vi "Log Status.vi"(7 "Context ID":u32, 8 "error in":errorcluster, 9 "Action":T1, 10 "Socket Counter":u32, 11 "Context Counter":u32) -> (0 "error out":errorcluster)   [LabVIEW 2019, in "RemoteControl.ZMQ.lvlib" / "ZMQ.ContextManager.lvlib"]
uses:
  ZMQ.ContextManager.lvlib
  Typedefs/Action--enum.ctl
  <vilib>/Utility/sysdir.llb/System Directory Type.ctl
  <vilib>/Utility/file.llb/Write Delimited Spreadsheet (string).vi
  <vilib>/Utility/config.llb/Read Key (Boolean).vi
  <vilib>/Utility/config.llb/Write Key (Boolean).vi
  <vilib>/Utility/config.llb/NI_LVConfig.lvlib
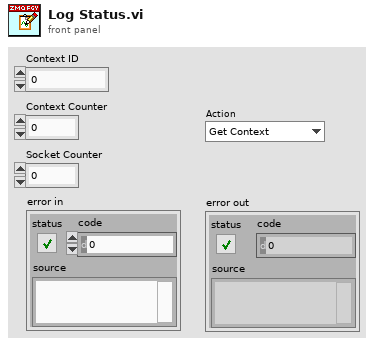
[diagram p1: front panel]
types:
  T1 = typedef "RemoteControl.ZMQ.lvlib/ZMQ.ContextManager.lvlib/Action--enum.ctl" = enum16{"Get Context", "Release Context", "Socket Opened", "Socket Closed", "Force Cleanup", "Set Context", "Retire If Idle"}
  T2 = typedef "System Directory Type.ctl" = i32
  T3 = typedef "NI_LVConfig.lvlib/Config Data RefNum.ctl" = refnum<k1>
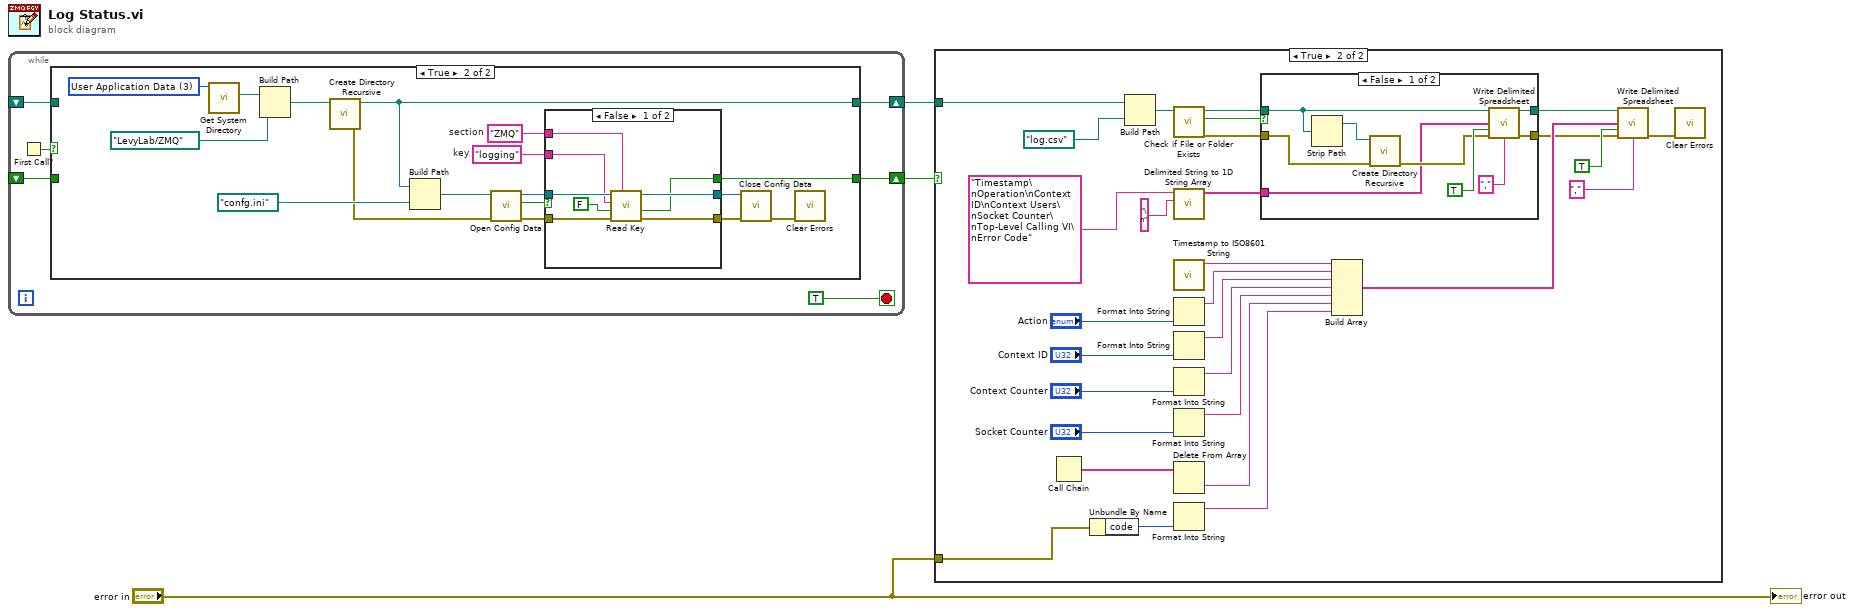
[diagram p0: block diagram]
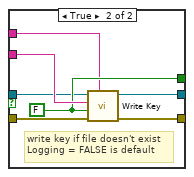
[diagram p3: hidden frame]
diagram:
  n1 = while {
    shift-right: [w8] -> w2
    shift-left: _ -> [w5]
    shift-right: [w9] -> w3
    shift-left: _ -> [w6]
    stop <- TRUE stop-if-true
    n2 = First Call?() -> (First Call?: T/F=w4:bool)
    n3 = case shown="True" w4 {
      tunnel: [w11 w19] -> w9
      tunnel: [w10 w14] -> w8
      tunnel: w6 -> [w11 _]
      tunnel: w5 -> [w10 _]
      frame False {
      }
      frame True {
        w16 = "logging"  # key
        w17 = "ZMQ"  # section
        w28 = T2 3 items=["User Home"=0, "User Desktop"=1, "User Documents"=2, "User Application Data"=3, "User Preferences"=4, "User Temporary"=5, "Public Documents"=6, "Public Application Data"=7, "Public Preferences"=8, "Public Cache"=13, "System Core Libraries"=9, "System Installed Libraries"=10, "Application Files"=11, "Boot Volume Root"=12] ("system directory type")
        n4 = call <vilib>:"Get System Directory.vi"("system directory type"=w28) -> ("system directory"=w27:path)  [unwired: 10 in]
        n5 = Build Path(base path=w27, name or relative path=path "LevyLab/ZMQ") -> (appended path=w15:path)
        n6 = call <vilib>:"Create Directory Recursive.vi"("directory"=w15) -> ("error out"=w13:errorcluster, "directory copy"=w14:path)  [unwired: 4 in, 1 out]
        n7 = Build Path(base path=w14, name or relative path=path "confg.ini") -> (appended path=w24:path)
        n8 = call <vilib>:"Open Config Data.vi"("error in (no error)"=w13, "configuration file path"=w24) -> ("error out"=w22:errorcluster, "file created?"=w18:bool, "refnum"=w23:T3)  [unwired: 7 in]
        n9 = case shown="False" w18 {
          tunnel: w23 -> [w36 w38]
          tunnel: w22 -> [w35 w37]
          tunnel: [w33 w41] -> w21
          tunnel: [w32 w40] -> w20
          tunnel: [w31 w42] -> w19
          tunnel: w17 -> [w30 w39]
          tunnel: w16 -> [w29 w43]
          frame False {
            n10 = call-poly <vilib>:"Read Key.vi"("section"=w30, "error in (no error)"=w35, "default value"=FALSE, "key"=w29, "refnum"=w36) -> ("error out"=w32:errorcluster, "value"=w31:bool, "refnum out"=w33:T3)  [unwired: 3 in, 1 out]
          }
          frame True {
            w42 = FALSE ("value")
            # "write key if file doesn't exist\nLogging = FALSE is default"
            n11 = call-poly <vilib>:"Write Key.vi"("section"=w39, "error in (no error)"=w37, "value"=w42, "key"=w43, "refnum"=w38) -> ("error out"=w40:errorcluster, "refnum out"=w41:T3)  [unwired: 4 in, 1 out]
          }
        }
        n12 = call <vilib>:"Close Config Data.vi"("error in (no error)"=w20, "refnum"=w21) -> ("error out"=w12:errorcluster)  [unwired: 8 in, 1 out]
        n13 = call <vilib>:"Clear Errors.vi"("error in (no error)"=w12) -> ()  [unwired: 5 in, 2 out]
      }
    }
  }
  n14 = case shown="True" w3 {
    tunnel: "error in" -> [_ w45]
    tunnel: w2 -> [_ w46]
    frame False {
    }
    frame True {
      n15 = Call Chain() -> (call chain=w56:string[])
      n16 = Unbundle By Name(w45) -> ("code"=w61:i32)
      n17 = Build Path(base path=w46, name or relative path=path "log.csv") -> (appended path=w47:path)
      n18 = call <vilib>:"Check if File or Folder Exists.vi"("path"=w47) -> ("error out"=w62:errorcluster, "file or folder exists?"=w69:bool, "dup path"=w70:path)  [unwired: 8 in]
      n19 = call <vilib>:"Delimited String to 1D String Array.vi"("delimiter"="\n", "delimited string"="Timestamp\nOperation\nContext ID\nContext Users\nSocket Counter\nTop-Level Calling VI\nError Code") -> ("string array"=w71:string[])  [unwired: 9 in]
      n20 = call <vilib>:"Timestamp to ISO8601 String.vi"() -> ("ISO8601 String"=w68:string)  [unwired: 11 in]
      n21 = Format Into String("Action") -> (resulting string=w49:string)  [unwired: 3 in, 1 out]
      n22 = Format Into String("Context ID") -> (resulting string=w50:string)  [unwired: 3 in, 1 out]
      n23 = Format Into String("Context Counter") -> (resulting string=w51:string)  [unwired: 3 in, 1 out]
      n24 = Format Into String("Socket Counter") -> (resulting string=w53:string)  [unwired: 3 in, 1 out]
      n25 = Delete From Array(array=w56) -> (deleted portion=w57:string)  [unwired: 2 in, 1 out]
      n26 = Format Into String(w61) -> (resulting string=w60:string)  [unwired: 3 in, 1 out]
      n27 = case shown="False" w69 {
        tunnel: w71 -> [w73 _]
        tunnel: w70 -> [w78 w82]
        tunnel: [w80 w82] -> w65
        tunnel: [w79 w83] -> w63
        tunnel: w62 -> [w75 w83]
        frame False {
          n28 = Strip Path(path=w78) -> (stripped path=w77:path)  [unwired: 1 out]
          n29 = call <vilib>:"Create Directory Recursive.vi"("error in (no error)"=w75, "directory"=w77) -> ("error out"=w74:errorcluster)  [unwired: 3 in, 2 out]
          n30 = call-poly <vilib>:"Write Delimited Spreadsheet.vi"("file path (dialog if empty)"=w78, "1D data"=w73, "append to file? (new file:F)"=TRUE, "error in (no error)"=w74, "delimiter (\\t)"="," ("delimiter (\\t)")) -> ("new file path (Not A Path if cancelled)"=w80:path, "error out"=w79:errorcluster)  [unwired: 9 in]
        }
        frame True {
        }
      }
      n31 = Build Array(w68, w49, w50, w51, w53, w57, w60) -> (w64:string[])
      n32 = call-poly <vilib>:"Write Delimited Spreadsheet.vi"("file path (dialog if empty)"=w65, "1D data"=w64, "append to file? (new file:F)"=TRUE, "error in (no error)"=w63, "delimiter (\\t)"="," ("delimiter (\\t)")) -> ("error out"=w44:errorcluster)  [unwired: 9 in, 1 out]
      n33 = call <vilib>:"Clear Errors.vi"("error in (no error)"=w44) -> ()  [unwired: 5 in, 2 out]
    }
  }
  "error out" <- "error in"
